vi "Write Outputs.vi"(8 "error in (no error)":errorcluster, 11 "Modbus in":refnum<class "Modbus.lvclass">) -> (0 "error out":errorcluster, 3 "Modbus out":refnum<class "Modbus.lvclass">)   [LabVIEW 2026, in "Modbus.lvlib" / "Modbus.lvclass"]
uses:
  Modbus.lvclass
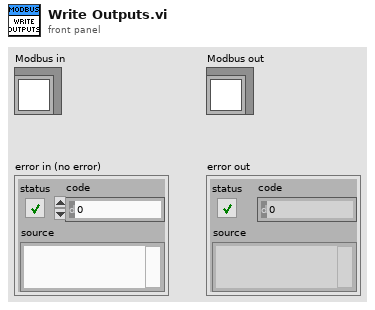
[diagram p1: front panel]
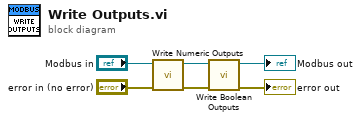
[diagram p0: block diagram]
diagram:
  n1 = call "Write Numeric Outputs.vi"("error in (no error)"="error in (no error)", "Modbus in"="Modbus in") -> ("error out"=w2:errorcluster, "Modbus out"=w3:refnum<class "Modbus.lvclass">)  [unwired: 8 in]
  n2 = call "Write Boolean Outputs.vi"("error in (no error)"=w2, "Modbus in"=w3) -> ("error out"=→"error out":errorcluster, "Modbus out"=→"Modbus out":refnum<class "Modbus.lvclass">)  [unwired: 8 in]
